vi "static sheet (shared buffer).vi"() -> ()   [LabVIEW 2020]
uses:
  HW Timed SPIM/HW Timed SPIM/DAQ Timed SPIM.lvclass
  C:/Program Files/National Instruments/LabVIEW 2020/vi.lib/ActorFramework/Actor/Actor.lvclass
  HW Timed SPIM/HamamatsuFluor_v2/HamamatsuFluor/HamamatsuFluor.lvclass
  C:/WormSPIM/Labview2/SPIM Engine/HW Timed SPIM/Abstract DAQ Triggered Actor/Abstract DAQ Triggered Actor.lvclass
  HW Timed SPIM/DAQ Timed SPIM Messages/Add Camera Msg/Add Camera Msg.lvclass/Add Camera Msg.ctl
  <vilib>/ActorFramework/Message Enqueuer/Message Enqueuer.lvclass/Message Enqueuer.ctl
  <vilib>/ActorFramework/Reply Msg/Reply Msg.lvclass/Reply Msg.ctl
  HW Timed SPIM/HamamatsuFluor_v2/HamamatsuFluor Messages/Set Sensor Mode Msg/Set Sensor Mode Msg.lvclass/Set Sensor Mode Msg.ctl
  HW Timed SPIM/HamamatsuFluor_v2/HamamatsuFluor Messages/Set ROI v2 Msg/Set ROI v2 Msg.lvclass/Set ROI v2 Msg.ctl
  HW Timed SPIM/HamamatsuFluor_v2/HamamatsuFluor Messages/Set Buffer Length Msg/Set Buffer Length Msg.lvclass/Set Buffer Length Msg.ctl
  HW Timed SPIM/Abstract DAQ Triggered Actor Messages/Set Save Directory Msg/Set Save Directory Msg.lvclass/Set Save Directory Msg.ctl
  HW Timed SPIM/DAQ Timed SPIM Messages/Set Main Loop Data Msg/Set Main Loop Data Msg.lvclass/Set Main Loop Data Msg.ctl
  HW Timed SPIM/DAQ Timed SPIM Messages/Set Warmup Data Msg/Set Warmup Data Msg.lvclass/Set Warmup Data Msg.ctl
  HW Timed SPIM/DAQ Timed SPIM Messages/Set Cooldown Data Msg/Set Cooldown Data Msg.lvclass/Set Cooldown Data Msg.ctl
  <vilib>/ActorFramework/Message Enqueuer/Enqueue.vi
  <vilib>/ActorFramework/Reply Msg/Send Message And Wait For Response.vi
  HW Timed SPIM/DAQ Timed SPIM Messages/Add Camera Msg/Add Camera Msg.lvclass
  C:/Program Files/National Instruments/LabVIEW 2020/vi.lib/ActorFramework/Message/Message.lvclass
  HW Timed SPIM/DAQ Timed SPIM Messages/Get Device Enqueuers Msg/Get Device Enqueuers Msg.lvclass
  C:/Program Files/National Instruments/LabVIEW 2020/vi.lib/ActorFramework/Reply Msg/Reply Msg.lvclass
  <vilib>/ActorFramework/Reply Msg/Reply Msg.lvclass
  HW Timed SPIM/HamamatsuFluor_v2/HamamatsuFluor Messages/Set Sensor Mode Msg/Set Sensor Mode Msg.lvclass
  HW Timed SPIM/HamamatsuFluor_v2/HamamatsuFluor Messages/Set ROI v2 Msg/Set ROI v2 Msg.lvclass
  HW Timed SPIM/HamamatsuFluor_v2/HamamatsuFluor Messages/Set Buffer Length Msg/Set Buffer Length Msg.lvclass
  HW Timed SPIM/Abstract DAQ Triggered Actor Messages/Set Save Directory Msg/Set Save Directory Msg.lvclass
  HW Timed SPIM/DAQ Timed SPIM Messages/Launch Basic Controller Msg/Launch Basic Controller Msg.lvclass
  <vilib>/ActorFramework/Stop Msg/Stop Msg.lvclass
  HW Timed SPIM/DAQ Timed SPIM Messages/Set Main Loop Data Msg/Set Main Loop Data Msg.lvclass
  HW Timed SPIM/DAQ Timed SPIM Messages/Set Warmup Data Msg/Set Warmup Data Msg.lvclass
  HW Timed SPIM/DAQ Timed SPIM Messages/Set Cooldown Data Msg/Set Cooldown Data Msg.lvclass
  <vilib>/ActorFramework/Message Priority Queue/Priority Enqueue.vi
  <vilib>/ActorFramework/Message Enqueuer/Message Enqueuer.lvclass
  <vilib>/ActorFramework/Actor/Actor.lvclass
  <resource>/objmgr/daqmx.rc
  Scan generators/Scan Generators.lvlib
panel:
  out "error out":errorcluster
  in  "error in (no error)":errorcluster
  in  "Z Slices":cluster{"start":dbl, "delta":dbl, "end":dbl}={"start"=100.0, "delta"=-1.355, "end"=20.0}
  in  "Signal delays":T1={"ETL delay (samples)"=10, "Scanner delay (samples)"=-25, "Laser delay (samples)"=2}
  in  "Volume period (s)":dbl=0.1
  in  "Frame period (s)":dbl=0.0015
  in  "Laser exposure (s)":dbl=0.00025
  in  "Scanner calibration":cluster{"Offset":dbl, "Amplitude":dbl}[](array[cluster])=[{"Offset"=2.5, "Amplitude"=-0.31}, {"Offset"=2.5, "Amplitude"=0.0}, {"Offset"=2.5, "Amplitude"=0.0}, {"Offset"=2.5, "Amplitude"=0.0}] {"Amplitude" min=-5.0 max=5.0 step=0.005; "Offset" min=0.0 max=5.0 step=0.005}
  in  "ROI":T2={"Horizontal Offset"=256, "Vertical Offset"=896, "Horizontal Size"=1536, "Vertical Size"=256}
  in  "Path":path=path "E:/"
  in  "stop":bool
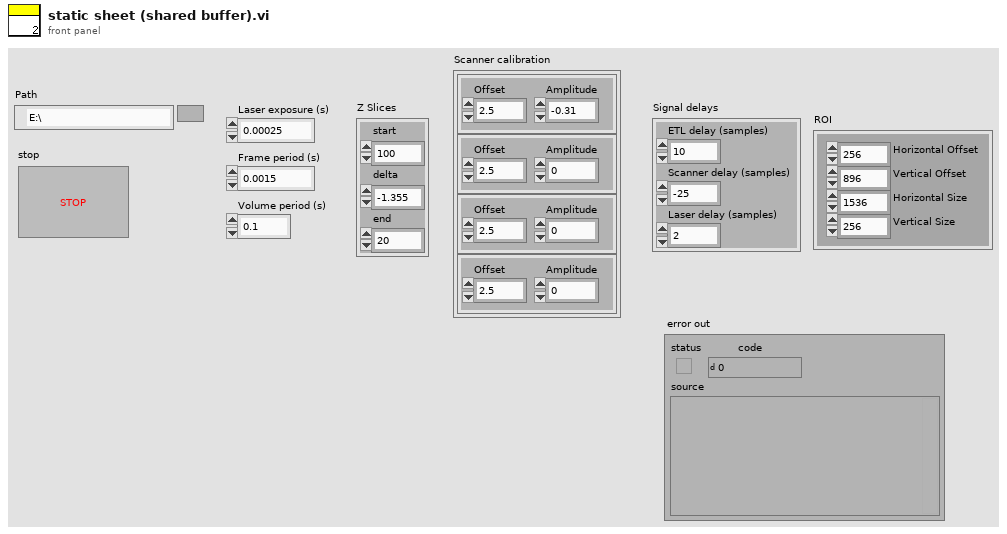
[diagram p1: front panel]
types:
  T1 = cluster{"ETL delay (samples)":i32, "Scanner delay (samples)":i32, "Laser delay (samples)":i32}
  T2 = cluster{"Horizontal Offset":i32, "Vertical Offset":i32, "Horizontal Size":i32, "Vertical Size":i32}
  T3 = enum16{"AREA", "DUAL LIGHT SHEET", "PROGRESSIVE"}
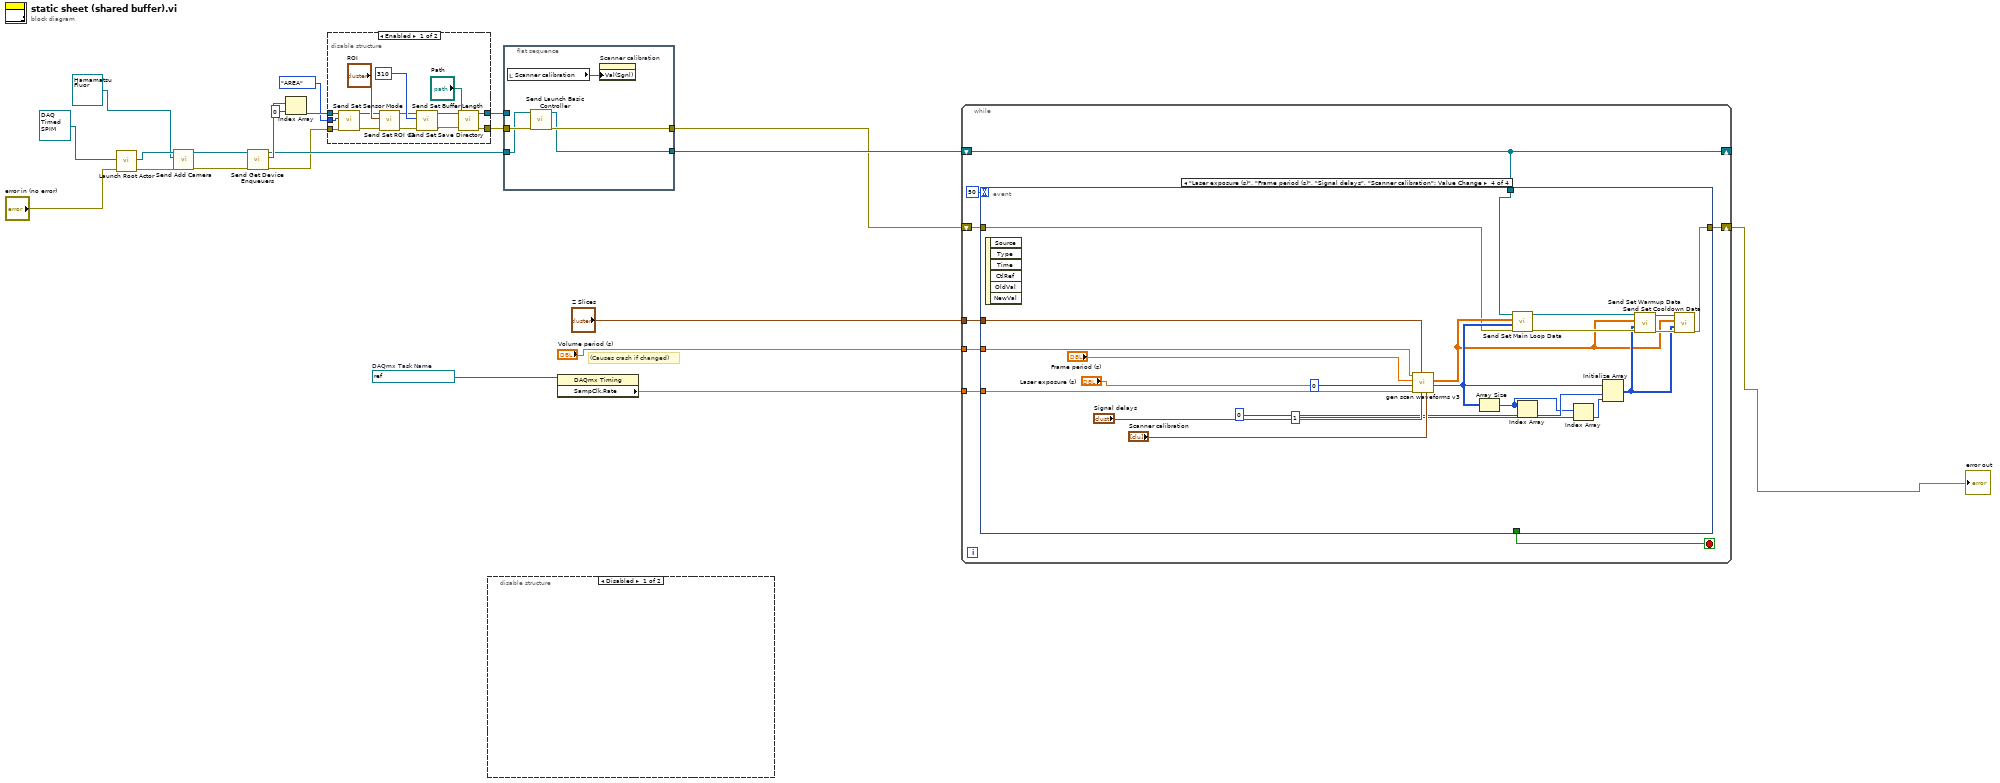
[diagram p0: block diagram]
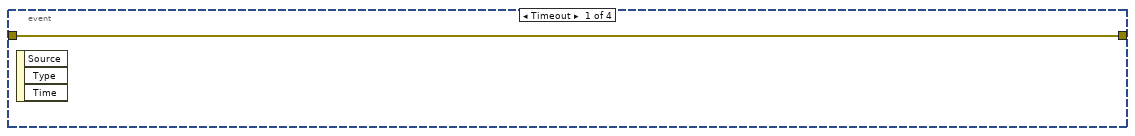
[diagram p4: hidden frame]
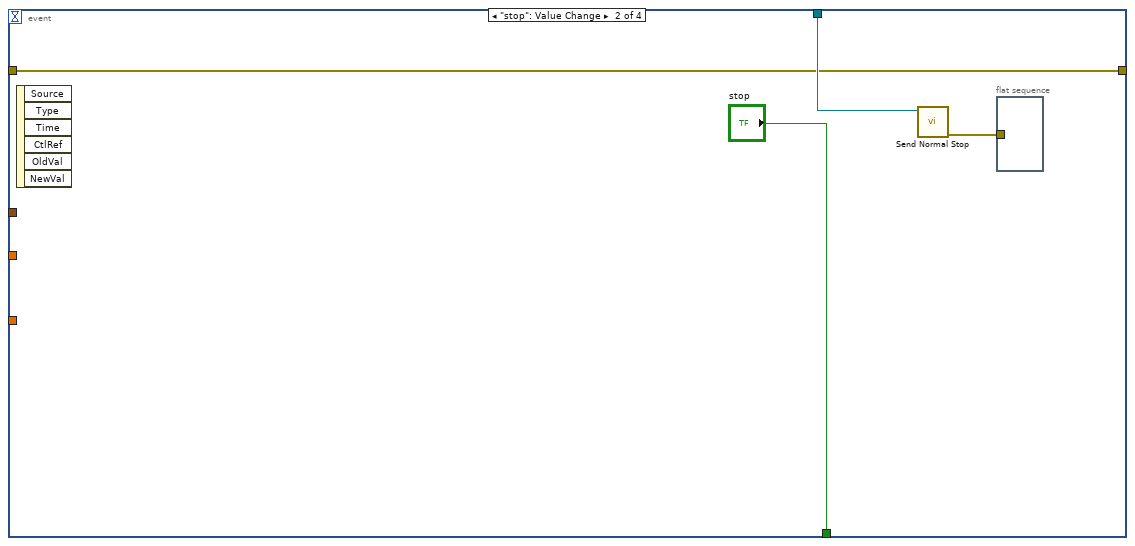
[diagram p5: hidden frame]
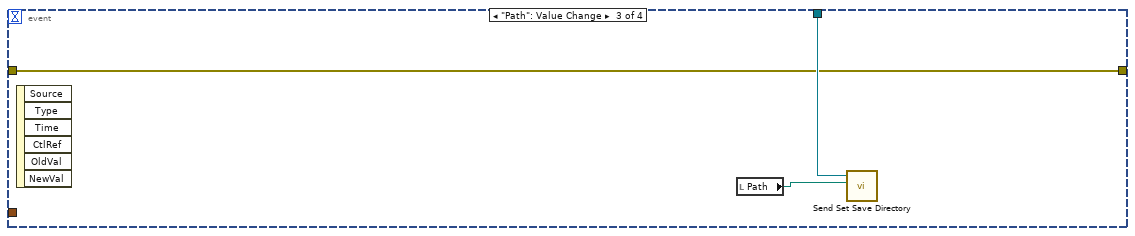
[diagram p6: hidden frame]
diagram:
  w19 = refnum<k21> "SPIM_Analog_Task"  # DAQmx Task Name
  # "(Causes crash if changed)"
  n1 = call <vilib>:"Launch Root Actor.vi"("error in (no error)"="error in (no error)", "Actor"=refnum<class "DAQ Timed SPIM.lvclass"> refnum ("DAQ Timed SPIM.lvlib:DAQ Timed SPIM.lvclass")) -> ("error out"=w20:errorcluster, "Actor's Enqueuer"=w21:refnum<class "Message Enqueuer.lvclass">)  [unwired: 8 in]
  n2 = call "Send Add Camera.vi"("error in (no error)"=w20, "DAQ Timed Camera"=refnum<class "HamamatsuFluor.lvclass"> refnum ("DAQ Timed SPIM.lvlib:HamamatsuFluor_v2.lvlib:HamamatsuFluor.lvclass"), "Message Enqueuer"=w21) -> ("error out"=w17:errorcluster, "Message Enqueuer out"=w18:refnum<class "Message Enqueuer.lvclass">)  [unwired: 7 in]
  n3 = call "Send Get Device Enqueuers.vi"("error in (no error)"=w17, "Message Enqueuer"=w18) -> ("error out"=w4:errorcluster, "Camera Enqueuers"=w16:refnum<class "Message Enqueuer.lvclass">[], "Message Enqueuer out"=w11:refnum<class "Message Enqueuer.lvclass">)  [unwired: 6 in, 1 out]
  n4 = Index Array(array=w16, index=0) -> (element=w5:refnum<class "Message Enqueuer.lvclass">)
  n5 = disable-structure shown="Enabled" {
    disable-tunnel: [w36 w37] -> w7
    disable-tunnel: [w35 w38] -> w6
    disable-tunnel: w5 -> [w33 w38]
    disable-tunnel: w4 -> [w32 w37]
    disable-tunnel: T3."AREA" ("Enum") -> [w23 _]
    frame Enabled {
      n6 = call "Send Set Sensor Mode.vi"("error in (no error)"=w32, "Enum"=w23, "Message Enqueuer"=w33) -> ("error out"=w29:errorcluster, "Message Enqueuer out"=w30:refnum<class "Message Enqueuer.lvclass">)  [unwired: 7 in]
      n7 = call "Send Set ROI v2.vi"("error in (no error)"=w29, "ROI"="ROI", "Message Enqueuer"=w30) -> ("error out"=w26:errorcluster, "Message Enqueuer out"=w27:refnum<class "Message Enqueuer.lvclass">)  [unwired: 7 in]
      n8 = call "Send Set Buffer Length.vi"("error in (no error)"=w26, "Buffer Size"=310, "Message Enqueuer"=w27) -> ("error out"=w24:errorcluster, "Message Enqueuer out"=w25:refnum<class "Message Enqueuer.lvclass">)  [unwired: 7 in]
      n9 = call "Send Set Save Directory.vi"("error in (no error)"=w24, "Path"="Path", "Message Enqueuer"=w25) -> ("error out"=w36:errorcluster, "Message Enqueuer out"=w35:refnum<class "Message Enqueuer.lvclass">)  [unwired: 7 in]
    }
    frame Disabled {
    }
  }
  n10 = disable-structure shown="Disabled" {
    frame Disabled {
    }
    frame Enabled {
    }
  }
  n11 = flat-sequence {
    tunnel: w7 -> [w42]
    tunnel: [w41] -> w3
    tunnel: w6 -> [_]
    tunnel: w11 -> [w40]
    tunnel: [w39] -> w10
    frame #0 {
      n12 = local read "Scanner calibration"() -> (w43:cluster{"Offset":dbl, "Amplitude":dbl}[])
      n13 = call "Send Launch Basic Controller.vi"("error in (no error)"=w42, "Message Enqueuer"=w40) -> ("error out"=w41:errorcluster, "Message Enqueuer out"=w39:refnum<class "Message Enqueuer.lvclass">)  [unwired: 8 in]
      n14 = property on="Scanner calibration" class="Arr (strict)"("Val(Sgnl)"=w43) -> ()  [unwired: 2 in, 2 out]
    }
  }
  n15 = property class="DAQmx Timing"(reference=w19) -> ("SampClk.Rate"=w14:dbl)  [unwired: 1 in, 2 out]
  n16 = while {
    shift-right: [w50] -> _
    shift-left: w10 -> [w50]
    tunnel: w14 -> [w49]
    tunnel: "Z Slices" -> [w48]
    tunnel: "Volume period (s)" -> [w47]
    shift-right: [w44] -> w2
    shift-left: w3 -> [w45]
    stop <- w51 stop-if-true
    n17 = event shown="[3] \"Laser exposure (s)\", \"Frame period (s)\", \"Signal delays\", \"Scanner calibration\": Value Change" {
      selector: _ -> [_ _ _ _]
      dyn-events: _ -> [_ _ _ _]
      timeout: 50 -> [_ _ _ _]
      tunnel: [_ "stop" _ _] -> w51
      tunnel: w50 -> [_ w55 w59 w69]
      tunnel: w49 -> [_ _ _ w72]
      tunnel: w48 -> [_ _ _ w63]
      tunnel: w47 -> [_ _ _ w62]
      tunnel: w45 -> [w52 w53 w57 w61]
      tunnel: [w52 w53 w57 w60] -> w44
      event Timeout {
        n18 = event-data() -> ()  [unwired: 1 in, 3 out]
      }
      event "stop": Value Change {
        n19 = event-data() -> ()  [unwired: 1 in, 6 out]
        n20 = call <vilib>:"Send Normal Stop.vi"("Message Enqueuer"=w55) -> ("error out"=w54:errorcluster)  [unwired: 10 in]
        n21 = flat-sequence {
          tunnel: w54 -> [_]
          frame #0 {
          }
        }
      }
      event "Path": Value Change {
        n22 = event-data() -> ()  [unwired: 1 in, 6 out]
        n23 = local read "Path"() -> (w58:path)
        n24 = call "Send Set Save Directory.vi"("Path"=w58, "Message Enqueuer"=w59) -> ()  [unwired: 8 in, 2 out]
      }
      event "Laser exposure (s)", "Frame period (s)", "Signal delays", "Scanner calibration": Value Change {
        n25 = event-data() -> ()  [unwired: 1 in, 6 out]
        n26 = call "gen scan waveforms v3.vi"("Scanner calibration"="Scanner calibration", "Signal delays"="Signal delays", "Z Slices"=w63, "AO sample rate"=w72, "Flash duration (s)"="Laser exposure (s)", "frame period (s)"="Frame period (s)", "volume period (s)"=w62) -> ("Digital signals"=w68:u8[][], "Analog signals"=w64:dbl[][])  [unwired: 3 in]
        n27 = Array Size(array=w68) -> (size(s)=w75:i32[])
        n28 = call "Send Set Main Loop Data.vi"("error in (no error)"=w61, "Digital"=w68, "Analog"=w64, "Message Enqueuer"=w69) -> ("error out"=w66:errorcluster, "Message Enqueuer out"=w67:refnum<class "Message Enqueuer.lvclass">)  [unwired: 6 in]
        n29 = Index Array(array=w75, index=0) -> (element=w76:i32)
        n30 = Index Array(array=w75, index=1) -> (element=w73:i32)
        n31 = Initialize Array(u8 0, w76, w73) -> (w65:u8[][])
        n32 = call "Send Set Warmup Data.vi"("error in (no error)"=w66, "Digital"=w65, "Analog"=w64, "Message Enqueuer"=w67) -> ("error out"=w70:errorcluster, "Message Enqueuer out"=w71:refnum<class "Message Enqueuer.lvclass">)  [unwired: 6 in]
        n33 = call "Send Set Cooldown Data.vi"("error in (no error)"=w70, "Digital"=w65, "Analog"=w64, "Message Enqueuer"=w71) -> ("error out"=w60:errorcluster)  [unwired: 6 in, 1 out]
      }
    }
  }
  "error out" <- w2
